vi "PicoLogCM3Example.vi"() -> ()   [LabVIEW 2016]
uses:
  PLCM3.dll
panel:
  out "Chan2 Value":dbl(knob) scale=0.0..100.0
  out "Chan1 Value":dbl(knob) min=0.0 max=10.0 scale=0.0..1000.0
  out "Chan3 Value":dbl(knob) scale=0.0..1000000.0
  out "Start time":timestamp
  out "UnitInfo fields":string[](array[string])=["Driver Version", "USB Version", "Hardware Version", "Variant Info", "Cal Date", "Kernal Driver Version"]
  out "UnitInfo":string[](array[string])
  out "End time":timestamp
  in  "Update settings":bool
  out "error out":errorcluster
  in  "IP Address:port number":string="192.168.1.30:6250"
  in  "Serial Number":string
  in  "Open by\nSerial Number":bool
  out "PLCM3 Units":string
  out "serialLth":u32
  in  "Enumerate USB/Ethernet/ALL":u32(ring)=4294967295 items=["USB"=1, "Ethernet"=2, "ALL"=4294967295]
  in  "error in (no error)":errorcluster
  in  "Connection":bool=TRUE
  in  "Reconnect Error":bool
  in  "Stop":bool
  out "GetValue PICO_STATUS log":T1(array[cluster]) {"Hex" format="%8x"}
  in  "CH3 Measurement Type":i32(ring) items=["OFF", "1mV range (1mV/A)", "10mV range (10mV/A)", "100mV range (100mV/A)", "Voltage Input (uV)"]
  in  "CH2 Measurement Type":i32(ring) items=["OFF", "1mV range (1mV/A)", "10mV range (10mV/A)", "100mV range (100mV/A)", "Voltage Input (uV)"]
  in  "CH1 Measurement Type":i32(ring)=1 items=["OFF", "1mV range (1mV/A)", "10mV range (10mV/A)", "100mV range (100mV/A)", "Voltage Input (uV)"]
  # "USB"
  # "Ethernet"
  # "Channel 1"
  # "Channel 2"
  # "Channel 3"
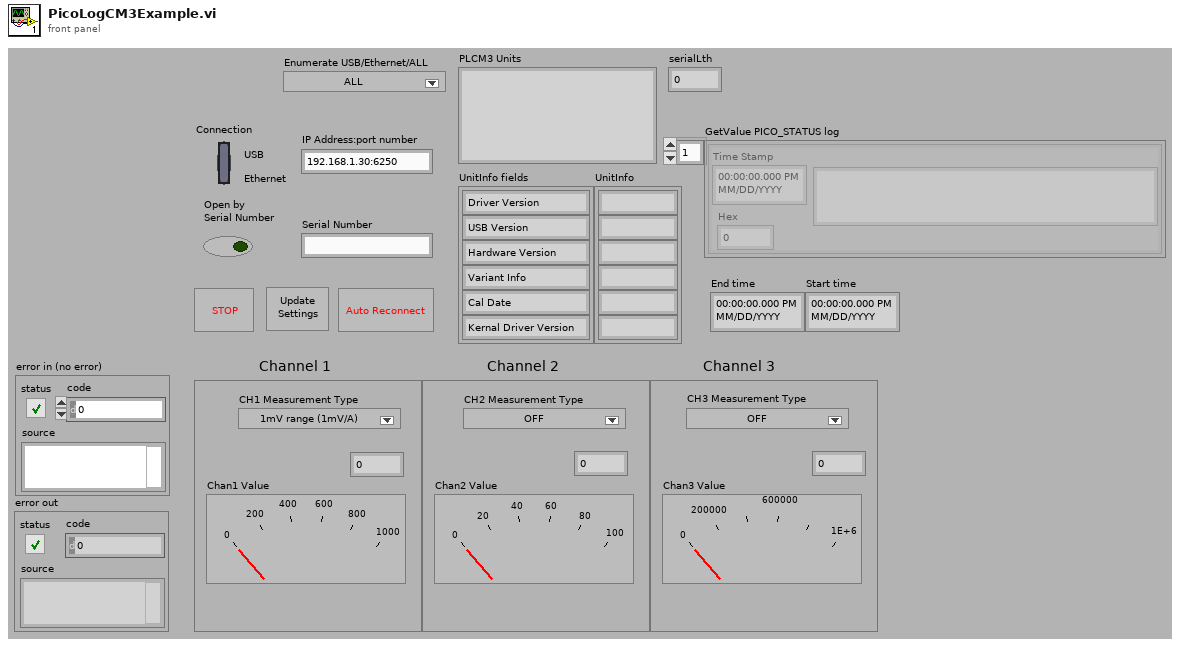
[diagram p1: front panel]
types:
  T1 = cluster{"Time Stamp":timestamp, "Hex":i32, "String":string}[]
  T2 = cluster{"seconds since 1Jan1904":timestamp, i32, "String":string}
  T3 = cluster{"seconds since 1Jan1904":timestamp, i32, "String":string}[]
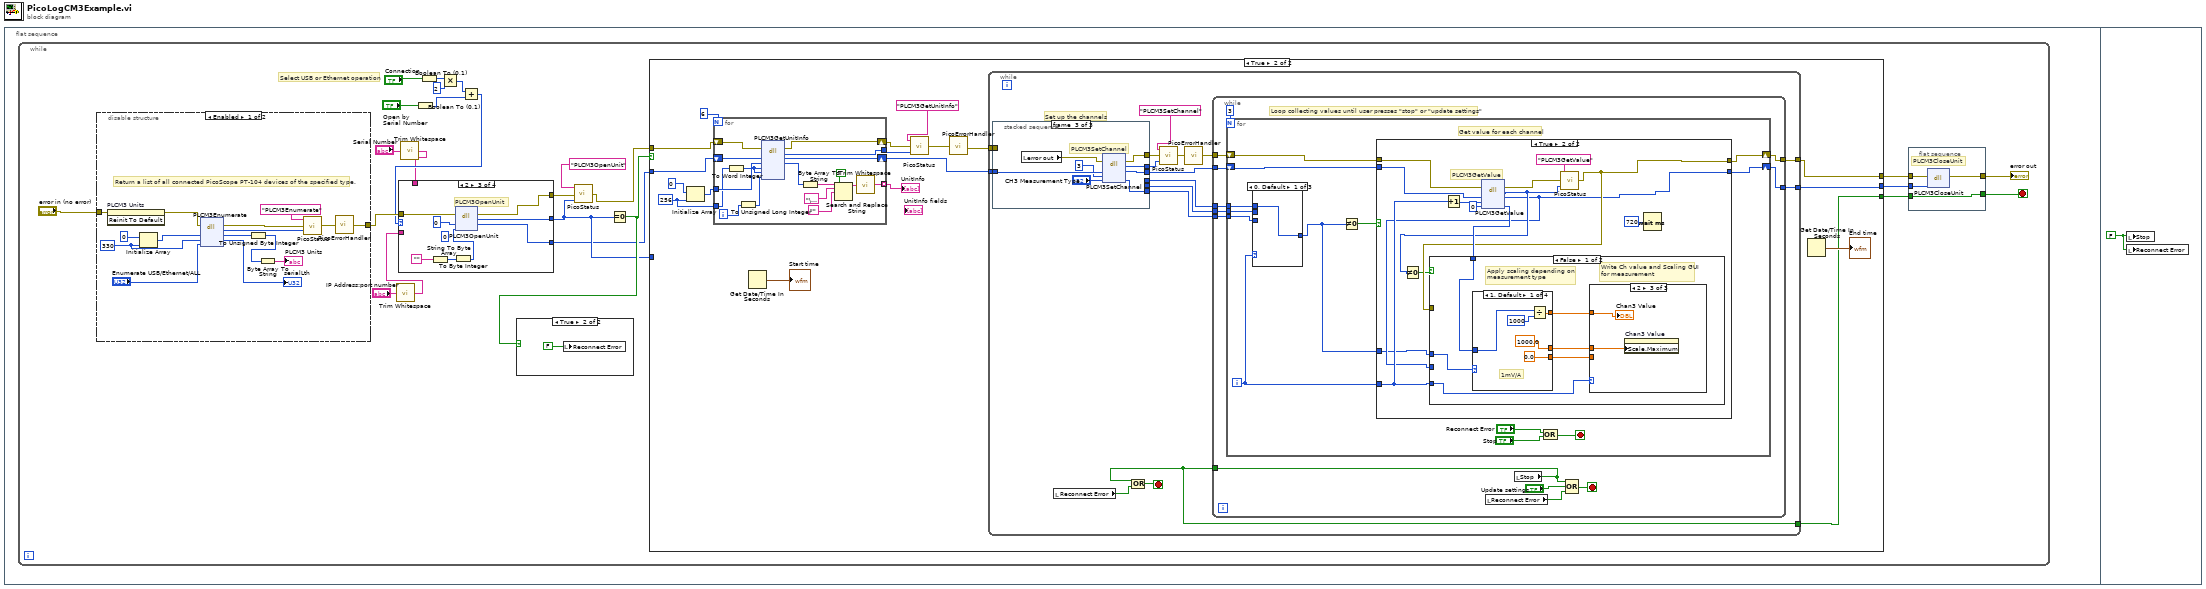
[diagram p0: block diagram]
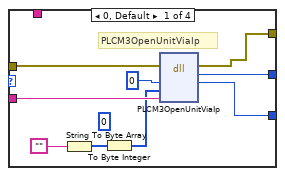
[diagram p4: hidden frame]
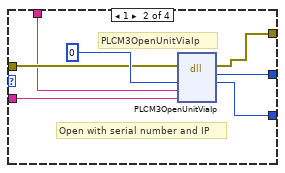
[diagram p5: hidden frame]
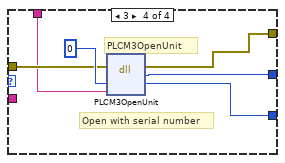
[diagram p6: hidden frame]
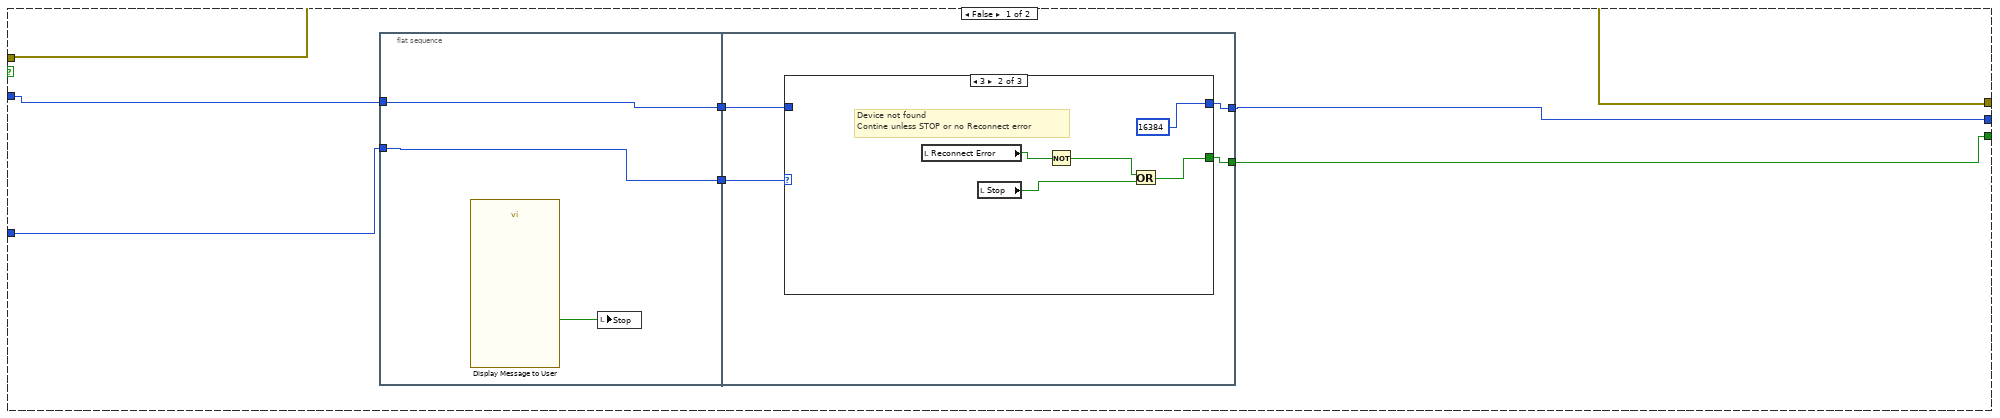
[diagram p7: hidden frame]
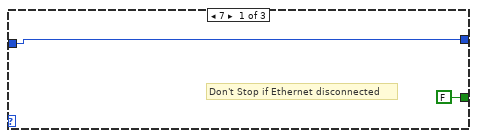
[diagram p8: hidden frame]
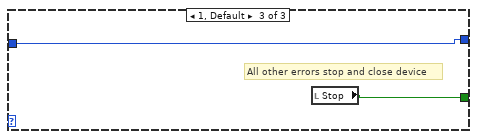
[diagram p9: hidden frame]
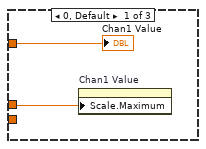
[diagram p11: hidden frame]
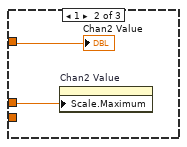
[diagram p12: hidden frame]
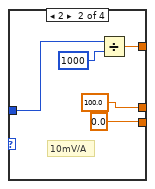
[diagram p13: hidden frame]
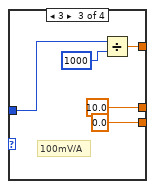
[diagram p14: hidden frame]
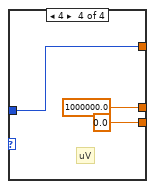
[diagram p15: hidden frame]
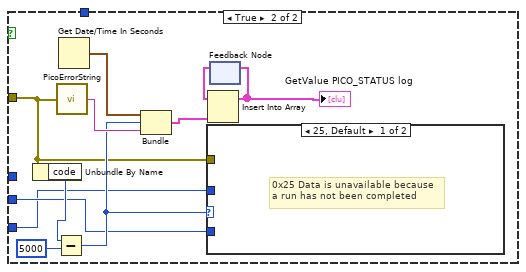
[diagram p16: hidden frame]
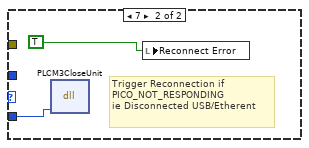
[diagram p17: hidden frame]
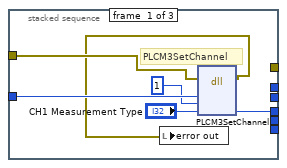
[diagram p20: hidden frame]
diagram:
  n1 = flat-sequence {
    frame #0 {
      n2 = while {
        stop <- w4 stop-if-true
        # "Select USB or Ethernet operation"
        n3 = disable-structure shown="Enabled" {
          disable-tunnel: [w28 w41] -> w19
          disable-tunnel: "error in (no error)" -> [w29 w41]
          frame Enabled {
            w33 = u32 330 ("dimension size")
            # "Return a list of all connected PicoScope PT-104 devices of the specified type."
            n4 = invoke on="PLCM3 Units" class="Str" method="Reinit To Default"(error in=w29) -> (error out=w30:errorcluster)  [unwired: 2 in, 2 out]
            n5 = Initialize Array(i8 0 ("U8"), w33) -> (w35:i8[])
            n6 = dll-call lib="PLCM3.dll" fn="PLCM3Enumerate"(error in=w30, "details_str"=w35, "length"=w33, "type"="Enumerate USB/Ethernet/ALL") -> (error out=w40:errorcluster, "PICO_STATUS"=w39:u32, "details_str"=w31:i8[], "length"=→"serialLth":u32)  [unwired: 3 in, 1 out]
            n7 = To Unsigned Byte Integer(number=w31) -> (unsigned 8bit integer=w32:u8[])
            n8 = Byte Array To String(unsigned byte array=w32) -> (string=→"PLCM3 Units":string)
            n9 = call "PicoStatus.vi"("PICO STATUS"=w39, "error in"=w40, "source"="PLCM3Enumerate") -> ("error out"=w27:errorcluster)
            n10 = call "PicoErrorHandler.vi"("error in"=w27) -> ("error out"=w28:errorcluster)
          }
          frame Disabled {
          }
        }
        n11 = call <vilib>:"Trim Whitespace.vi"("string"="IP Address:port number") -> ("trimmed string"=w8:string)  [unwired: 1 in]
        n12 = call <vilib>:"Trim Whitespace.vi"("string"="Serial Number") -> ("trimmed string"=w11:string)  [unwired: 1 in]
        n13 = Boolean To (0,1)(Boolean="Open by\nSerial Number") -> (0, 1=w13:i16)
        n14 = Boolean To (0,1)(Boolean="Connection") -> (0, 1=w16:i16)
        n15 = Multiply(x=w16, y=i16 2) -> (x*y=w14:i16)
        n16 = Add(x=w14, y=w13) -> (x+y=w12:i16)
        n17 = case shown="2" w12 {
          tunnel: [w50 w56 w65 w71] -> w3
          tunnel: [w49 w55 w63 w69] -> w2
          tunnel: [w48 w54 w64 w70] -> w21
          tunnel: w19 -> [w47 w53 w61 w67]
          tunnel: w11 -> [_ w52 _ w66]
          tunnel: w8 -> [w46 w51 _ _]
          frame 0, Default {
            (unwired) i8 0 ("handle")
            # "PLCM3OpenUnitViaIp"
            n18 = String To Byte Array(string="") -> (unsigned byte array=w44:u8[])
            n19 = To Byte Integer(number=w44) -> (8bit integer=w42:i8[])
            n20 = dll-call lib="PLCM3.dll" fn="PLCM3OpenUnitViaIp"(error in=w47, "handle"=i16 0, "serial"=w42, "IpAddress"=w46) -> (error out=w48:errorcluster, "Status"=w50:i32, "handle"=w49:i16)  [unwired: 4 in, 1 out]
          }
          frame 1 {
            # "Open with serial number and IP"
            # "PLCM3OpenUnitViaIp"
            n21 = dll-call lib="PLCM3.dll" fn="PLCM3OpenUnitViaIp"(error in=w53, "handle"=i16 0, "serial"=w52, "IpAddress"=w51) -> (error out=w54:errorcluster, "Status"=w56:i32, "handle"=w55:i16)  [unwired: 4 in, 1 out]
          }
          frame 2 {
            (unwired) i8 0 ("serial")
            # "PLCM3OpenUnit"
            n22 = String To Byte Array(string="") -> (unsigned byte array=w60:u8[])
            n23 = To Byte Integer(number=w60) -> (8bit integer=w58:i8[])
            n24 = dll-call lib="PLCM3.dll" fn="PLCM3OpenUnit"(error in=w61, "handle"=i16 0, "serial"=w58) -> (error out=w64:errorcluster, "Status"=w65:i32, "handle"=w63:i16)  [unwired: 3 in, 1 out]
          }
          frame 3 {
            # "Open with serial number"
            # "PLCM3OpenUnit"
            n25 = dll-call lib="PLCM3.dll" fn="PLCM3OpenUnit"(error in=w67, "handle"=i16 0, "serial"=w66) -> (error out=w70:errorcluster, "Status"=w71:i32, "handle"=w69:i16)  [unwired: 3 in, 1 out]
          }
        }
        n26 = call "PicoStatus.vi"("PICO STATUS"=w3, "error in"=w21, "source"="PLCM3OpenUnit") -> ("error out"=w1:errorcluster)
        n27 = Equal To 0?(x=w3) -> (x = 0?=w7:bool)
        n28 = case shown="True" w7 {
          frame False {
          }
          frame True {
            n29 = local write "Reconnect Error"(FALSE ("Stop 2")) -> ()
          }
        }
        n30 = case shown="True" w7 {
          tunnel: w2 -> [w80 w104]
          tunnel: [w78 w115] -> w24
          tunnel: [w79 w116] -> w23
          tunnel: w1 -> [w79 w105]
          tunnel: [w77 w103] -> w5
          tunnel: w3 -> [w76 _]
          frame False {
            n31 = flat-sequence {
              tunnel: w76 -> [w85]
              tunnel: [w85] -> w82
              tunnel: w80 -> [w84]
              tunnel: [w84] -> w81
              tunnel: [w89] -> w77
              tunnel: [w88] -> w78
              tunnel: w82 -> [w87]
              tunnel: w81 -> [w86]
              frame #0 {
                n32 = call "Display Message to User"() -> ("Stop"=w83:bool)  [unwired: 10 in, 1 out]
                n33 = local write "Stop"(w83) -> ()
              }
              frame #1 {
                n34 = case shown="3" w87 {
                  tunnel: [FALSE ("Stop") w94 w97] -> w89
                  tunnel: [w90 i16 16384 ("handle") w98] -> w88
                  tunnel: w86 -> [w90 _ w98]
                  frame 7 {
                    # "Don't Stop if Ethernet disconnected"
                  }
                  frame 3 {
                    # "Device not found\nContine unless STOP or no Reconnect error"
                    n35 = local read "Reconnect Error"() -> (w93:bool)
                    n36 = local read "Stop"() -> (w92:bool)
                    n37 = Not(x=w93) -> (.not. x?=w95:bool)
                    n38 = Or(x=w95, y=w92) -> (x .or. y?=w94:bool)
                  }
                  frame 1, Default {
                    # "All other errors stop and close device"
                    n39 = local read "Stop"() -> (w97:bool)
                  }
                }
              }
            }
          }
          frame True {
            w99 = 256 ("dimension size")
            n40 = Initialize Array(u8 0 ("element"), w99) -> (w111:u8[])
            n41 = for {
              N: 6 -> [_]
              tunnel: [w121] -> w110 mode=indexing
              tunnel: [w126] -> w113
              tunnel: w111 -> [w124]
              shift-right: [w127] -> w102
              shift-left: w104 -> [w129]
              shift-right: [w125] -> w112
              shift-left: w105 -> [w128]
              tunnel: w99 -> [w117]
              i -> [w119]
              n42 = To Word Integer(number=w117) -> (16bit integer=w118:i16)
              n43 = To Unsigned Long Integer(number=w119) -> (unsigned 32bit integer=w120:u32)
              n44 = dll-call lib="PLCM3.dll" fn="PLCM3GetUnitInfo"(error in=w128, "handle"=w129, "String"=w124, "StringLength"=w118, "requiredSize"=w118, "info"=w120) -> (error out=w125:errorcluster, "Status"=w126:i32, "handle"=w127:i16, "String"=w123:u8[])  [unwired: 5 in, 1 out]
              n45 = Byte Array To String(unsigned byte array=w123) -> (string=w122:string)
              n46 = Search and Replace String(replace all?=TRUE ("replace all? (F)"), input string=w122, search string="\u0000", replace string="") -> (result string=w130:string)  [unwired: 4 in, 3 out]
              n47 = call <vilib>:"Trim Whitespace.vi"("string"=w130) -> ("trimmed string"=w121:string)  [unwired: 1 in]
            }
            "UnitInfo" <- w110
            n48 = Get Date/Time In Seconds() -> (seconds since 1Jan1904=→"Start time":timestamp)
            n49 = call "PicoStatus.vi"("PICO STATUS"=w113, "error in"=w112, "source"="PLCM3GetUnitInfo") -> ("error out"=w100:errorcluster)
            n50 = call "PicoErrorHandler.vi"("error in"=w100) -> ("error out"=w101:errorcluster)
            n51 = while {
              tunnel: w102 -> [w149]
              tunnel: [w145] -> w115
              tunnel: [w144] -> w116
              tunnel: w101 -> [w143]
              tunnel: [w138] -> w103
              stop <- w140 stop-if-true
              # "Set up the channels"
              n52 = stacked-sequence {
                tunnel: w149 -> [w242 w248 w256]
                tunnel: [w239 _ _] -> w148
                tunnel: [_ w245 _] -> w147
                tunnel: [_ _ w253] -> w146
                tunnel: [_ _ w252] -> w136
                tunnel: [_ _ w251] -> w141
                tunnel: [_ _ w249] -> w137
                tunnel: w143 -> [w238 _ _]
                frame #0 {
                  # "PLCM3SetChannel"
                  n53 = dll-call lib="PLCM3.dll" fn="PLCM3SetChannel"(error in=w238, "handle"=w242, "channel"=1, "type"="CH1 Measurement Type") -> (error out=w237:errorcluster, "type"=w239:i32)  [unwired: 5 in, 1 out]
                  n54 = local write "error out"(w237) -> ()
                }
                frame #1 {
                  # "PLCM3SetChannel"
                  n55 = local read "error out"() -> (w243:errorcluster)
                  n56 = dll-call lib="PLCM3.dll" fn="PLCM3SetChannel"(error in=w243, "handle"=w248, "channel"=2, "type"="CH2 Measurement Type") -> (error out=w244:errorcluster, "type"=w245:i32)  [unwired: 5 in, 1 out]
                  n57 = local write "error out"(w244) -> ()
                }
                frame #2 {
                  # "PLCM3SetChannel"
                  n58 = local read "error out"() -> (w250:errorcluster)
                  n59 = dll-call lib="PLCM3.dll" fn="PLCM3SetChannel"(error in=w250, "handle"=w256, "channel"=3, "type"="CH3 Measurement Type") -> (error out=w251:errorcluster, "Status"=w249:i32, "handle"=w252:i16, "type"=w253:i32)  [unwired: 3 in, 1 out]
                }
              }
              n60 = local read "Reconnect Error"() -> (w139:bool)
              n61 = call "PicoStatus.vi"("PICO STATUS"=w137, "error in"=w141, "source"="PLCM3SetChannel") -> ("error out"=w134:errorcluster)
              n62 = call "PicoErrorHandler.vi"("error in"=w134) -> ("error out"=w135:errorcluster)
              n63 = while {
                tunnel: w148 -> [w161]
                tunnel: w147 -> [w160]
                tunnel: w146 -> [w159]
                tunnel: [w158] -> w145
                tunnel: [w152] -> w144
                tunnel: w136 -> [w151]
                tunnel: w135 -> [w156]
                tunnel: [w153] -> w138
                stop <- w155 stop-if-true
                # "Loop collecting values until user presses \"stop\" or \"update settings\""
                n64 = for {
                  N: 3 -> [_]
                  tunnel: w161 -> [w173]
                  tunnel: w160 -> [w174]
                  tunnel: w159 -> [w172]
                  shift-right: [w163] -> w152
                  shift-left: w156 -> [w168]
                  shift-right: [w169] -> w158
                  shift-left: w151 -> [w162]
                  i -> [w171]
                  stop <- w166 stop-if-true
                  # "Get value for each channel"
                  n65 = case shown="0, Default" w171 {
                    tunnel: [w234 w235 w236] -> w167
                    tunnel: w173 -> [w234 _ _]
                    tunnel: w174 -> [_ w235 _]
                    tunnel: w172 -> [_ _ w236]
                    frame 0, Default {
                    }
                    frame 1 {
                    }
                    frame 2 {
                    }
                  }
                  n66 = Not Equal To 0?(x=w167) -> (x != 0?=w170:bool)
                  n67 = case shown="True" w170 {
                    tunnel: w171 -> [_ w179]
                    tunnel: [w175 w178] -> w169
                    tunnel: [w176 w182] -> w163
                    tunnel: w168 -> [w176 w185]
                    tunnel: w162 -> [w175 w184]
                    tunnel: w167 -> [_ w177]
                    frame False {
                    }
                    frame True {
                      # "PLCM3GetValue"
                      n68 = Increment(x=w179) -> (x+1=w188:i32)
                      n69 = dll-call lib="PLCM3.dll" fn="PLCM3GetValue"(error in=w185, "handle"=w184, "channel"=w188, "value"=0) -> (error out=w189:errorcluster, "Status"=w180:i32, "handle"=w178:i16, "value"=w183:i32)  [unwired: 3 in, 1 out]
                      n70 = Not Equal To 0?(x=w180) -> (x != 0?=w181:bool)
                      n71 = call "PicoStatus.vi"("PICO STATUS"=w180, "error in"=w189, "source"="PLCM3GetValue") -> ("error out"=w182:errorcluster)
                      n72 = case shown="False" w181 {
                        tunnel: w182 -> [_ w221]
                        tunnel: w177 -> [w196 _]
                        tunnel: w183 -> [w195 _]
                        tunnel: w179 -> [w194 w222]
                        tunnel: w178 -> [_ w223]
                        frame False {
                          # "Write Ch value and Scaling GUI for measurement"
                          # "Apply scaling depending on \nmeasurement type"
                          n73 = case shown="1, Default" w196 {
                            tunnel: w195 -> [w206 w211 w216 w218]
                            tunnel: [w205 w210 w215 w218] -> w193
                            tunnel: [1000.0 ("Data Range:Maximum") 100.0 ("Data Range:Maximum") 10.0 ("Data Range:Maximum") 1000000.0 ("Data Range:Maximum")] -> w192
                            tunnel: [0.0 ("Scale.Range:Minimum") 0.0 ("Scale.Range:Minimum") 0.0 ("Scale.Range:Minimum") 0.0 ("Scale.Range:Minimum")] -> w191
                            frame 1, Default {
                              # "1mV/A"
                              n74 = Divide(x=w206, y=1000) -> (x/y=w205:dbl)
                            }
                            frame 2 {
                              # "10mV/A"
                              n75 = Divide(x=w211, y=1000) -> (x/y=w210:dbl)
                            }
                            frame 3 {
                              # "100mV/A"
                              n76 = Divide(x=w216, y=1000) -> (x/y=w215:dbl)
                            }
                            frame 4 {
                              # "uV"
                            }
                          }
                          n77 = case shown="2" w194 {
                            tunnel: w193 -> [w198 w200 w202]
                            tunnel: w192 -> [w197 w199 w201]
                            tunnel: w191 -> [_ _ _]
                            frame 0, Default {
                              n78 = property on="Chan1 Value" class="Knob (strict)"("Scale.Maximum"=w197) -> ()  [unwired: 2 in, 2 out]
                              "Chan1 Value" <- w198
                            }
                            frame 1 {
                              n79 = property on="Chan2 Value" class="Knob (strict)"("Scale.Maximum"=w199) -> ()  [unwired: 2 in, 2 out]
                              "Chan2 Value" <- w200
                            }
                            frame 2 {
                              n80 = property on="Chan3 Value" class="Knob (strict)"("Scale.Maximum"=w201) -> ()  [unwired: 2 in, 2 out]
                              "Chan3 Value" <- w202
                            }
                          }
                        }
                        frame True {
                          n81 = Unbundle By Name(w221) -> ("code"=w231:i32)
                          n82 = Subtract(x=w231, y=5000) -> (x-y=w224:i32)
                          n83 = call "PicoErrorString.vi"("error in"=w221) -> ("String"=w229:string)  [unwired: 2 in, 2 out]
                          n84 = Get Date/Time In Seconds() -> (seconds since 1Jan1904=w225:timestamp)
                          n85 = Bundle("seconds since 1Jan1904"=w225, w224, "String"=w229) -> (w228:T2)  [unwired: 1 in]
                          n86 = case shown="25, Default" w224 {
                            tunnel: w223 -> [_ w233]
                            tunnel: w222 -> [_ _]
                            tunnel: w221 -> [_ _]
                            frame 37, Default {
                              # "0x25 Data is unavailable because\na run has not been completed"
                            }
                            frame 7 {
                              # "Trigger Reconnection if\nPICO_NOT_RESPONDING\nie Disconnected USB/Etherent"
                              n87 = dll-call lib="PLCM3.dll" fn="PLCM3CloseUnit"("handle"=w233) -> ()  [unwired: 5 in, 2 out]
                              n88 = local write "Reconnect Error"(TRUE ("Stop 2")) -> ()
                            }
                          }
                          n89 = feedback #1() -> (w226:T3)  [unwired: 1 in]
                          n90 = Insert Into Array(array=w226, new element=w228) -> (w227:T3)  [unwired: 1 in]
                          "GetValue PICO_STATUS log" <- w227
                          n91 = feedback-in #1(w227) -> ()
                        }
                      }
                      n92 = Wait (ms)(milliseconds to wait=u32 720) -> ()  [unwired: 1 out]
                    }
                  }
                  n93 = Compound Arithmetic op=OR("Reconnect Error", "Stop") -> (w166:bool)
                }
                n94 = local read "Reconnect Error"() -> (w150:bool)
                n95 = local read "Stop"() -> (w153:bool)
                n96 = Compound Arithmetic op=OR(w153, "Update settings", w150) -> (w155:bool)
              }
              n97 = Compound Arithmetic op=OR(w138, w139) -> (w140:bool)
            }
            n98 = Get Date/Time In Seconds() -> (seconds since 1Jan1904=→"End time":timestamp)
          }
        }
        n99 = flat-sequence {
          tunnel: w24 -> [w75]
          tunnel: w23 -> [w74]
          tunnel: [w73] -> w6
          tunnel: w5 -> [w72]
          tunnel: [w72] -> w4
          frame #0 {
            # "PLCM3CloseUnit"
            n100 = dll-call lib="PLCM3.dll" fn="PLCM3CloseUnit"(error in=w74, "handle"=w75) -> (error out=w73:errorcluster)  [unwired: 4 in, 1 out]
          }
        }
        "error out" <- w6
      }
    }
    frame #1 {
      w257 = FALSE ("Stop")
      n101 = local write "Stop"(w257) -> ()
      n102 = local write "Reconnect Error"(w257) -> ()
    }
  }
